vi "Add Triggered Device.vi"(8 "error in (no error)":errorcluster, 10 "DAQ Timed Device":refnum<class "Abstract DAQ Triggered Actor.lvclass">, 11 "DAQ Timed SPIM in":refnum<class "DAQ Timed SPIM.lvclass">) -> (0 "error out":errorcluster, 3 "DAQ Timed SPIM out":refnum<class "DAQ Timed SPIM.lvclass">)   [LabVIEW 2020, in "DAQ Timed SPIM.lvlib" / "DAQ Timed SPIM.lvclass"]
uses:
  DAQ Timed SPIM.lvclass
  C:/Program Files/National Instruments/LabVIEW 2020/vi.lib/ActorFramework/Actor/Actor.lvclass
  Abstract DAQ Triggered Actor/Abstract DAQ Triggered Actor.lvclass
  DAQ Timed SPIM.lvclass/DAQ Timed SPIM.ctl
  <vilib>/ActorFramework/Actor/Actor.lvclass
  <vilib>/ActorFramework/Message Enqueuer/Message Enqueuer.lvclass
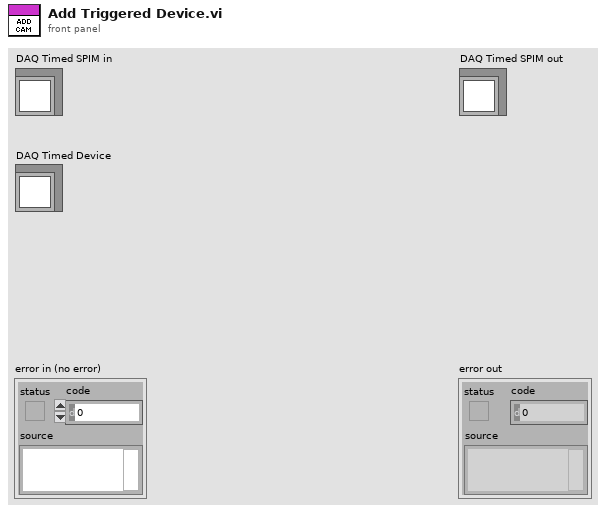
[diagram p1: front panel]
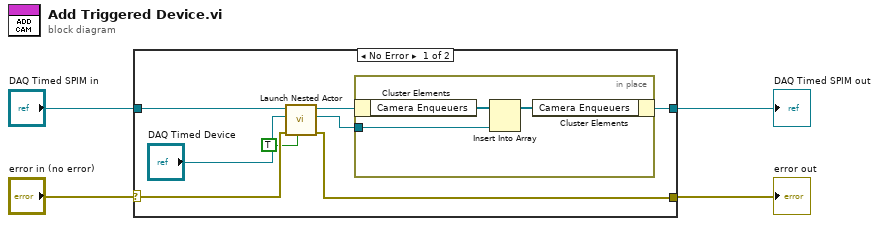
[diagram p0: block diagram]
diagram:
  n1 = case shown="No Error" "error in (no error)" {
    selector: "error in (no error)" -> [w7 w17]
    tunnel: [w6 w17] -> w3
    tunnel: [w9 w16] -> w1
    tunnel: "DAQ Timed SPIM in" -> [w12 w16]
    frame No Error {
      n2 = call <vilib>:"Launch Nested Actor.vi"("Open Actor Core front panel? (F)"=TRUE, "error in (no error)"=w7, "Nested Actor"="DAQ Timed Device", "Caller Actor in"=w12) -> ("error out"=w6:errorcluster, "Nested Actor's Enqueuer"=w8:refnum<class "Message Enqueuer.lvclass">, "Caller Actor out"=w10:refnum<class "DAQ Timed SPIM.lvclass">)  [unwired: 5 in]
      n3 = in-place {
        in-place-border: w8 -> [w13]
        n4 = in-place-cluster #1(w10) -> ("Camera Enqueuers"=w15:refnum<class "Message Enqueuer.lvclass">[])
        n5 = Insert Into Array(array=w15, new element=w13) -> (w14:refnum<class "Message Enqueuer.lvclass">[])  [unwired: 1 in]
        n6 = in-place-cluster #1("Camera Enqueuers"=w14) -> (w9:refnum<class "DAQ Timed SPIM.lvclass">)
      }
    }
    frame Error {
    }
  }
  "error out" <- w3
  "DAQ Timed SPIM out" <- w1
